vi "Get Cancellatioin Token.vi"(8 "error in (no error)":errorcluster caption="에러 입력(에러 없음)", 11 "Instrument Manager 입력":refnum<class "Instrument Manager.lvclass">) -> (0 "error out":errorcluster caption="에러 출력", 2 "Cancellation Token":refnum<notifier>, 3 "Instrument Manager 출력":refnum<class "Instrument Manager.lvclass">)   [LabVIEW 2023, in "Instrument Manager.lvclass"]
uses:
  Instrument Manager.lvclass
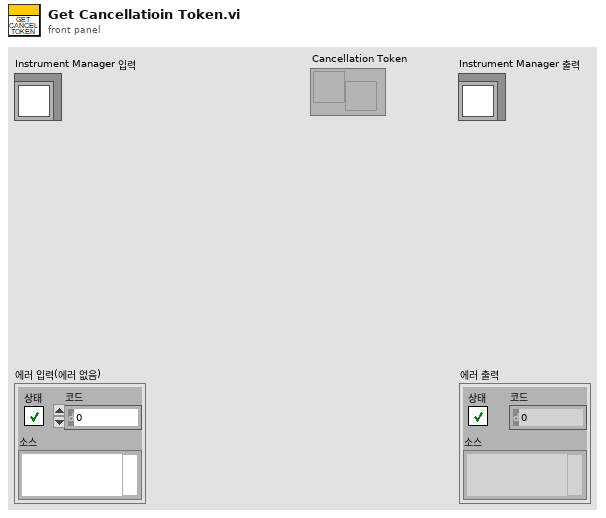
[diagram p1: front panel]
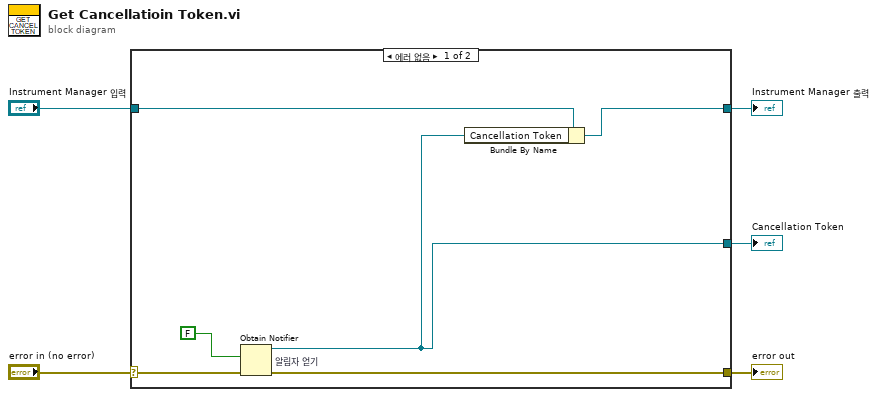
[diagram p0: block diagram]
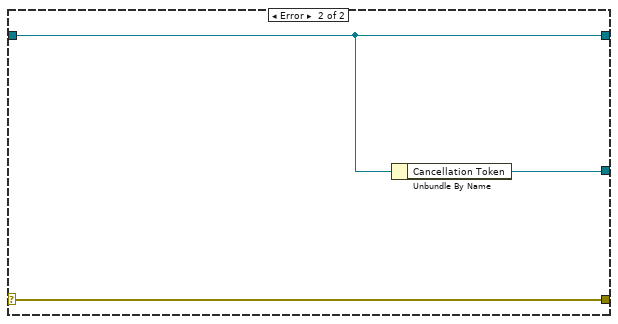
[diagram p2: hidden frame]
diagram:
  n1 = case shown="에러 없음" "error in (no error)" {
    selector: "error in (no error)" -> [w11 w14]
    tunnel: [w7 w14] -> w4
    tunnel: [w8 w13] -> w2
    tunnel: "Instrument Manager 입력" -> [w9 w13]
    tunnel: [w6 w12] -> w1
    frame No Error {
      n2 = Obtain Notifier "알림자 얻기"(notification data type=FALSE, error in (no error)=w11) -> (notifier out=w6:refnum<notifier>, error out=w7:errorcluster)  [unwired: 2 in, 1 out]
      n3 = Bundle By Name(cluster=w9, "Cancellation Token"=w6) -> (w8:refnum<class "Instrument Manager.lvclass">)
    }
    frame Error {
      n4 = Unbundle By Name(w13) -> ("Cancellation Token"=w12:refnum<notifier>)
    }
  }
  "error out" <- w4
  "Instrument Manager 출력" <- w2
  "Cancellation Token" <- w1
